vi "Sous_VI_recule.vi"   [LabVIEW 2017]
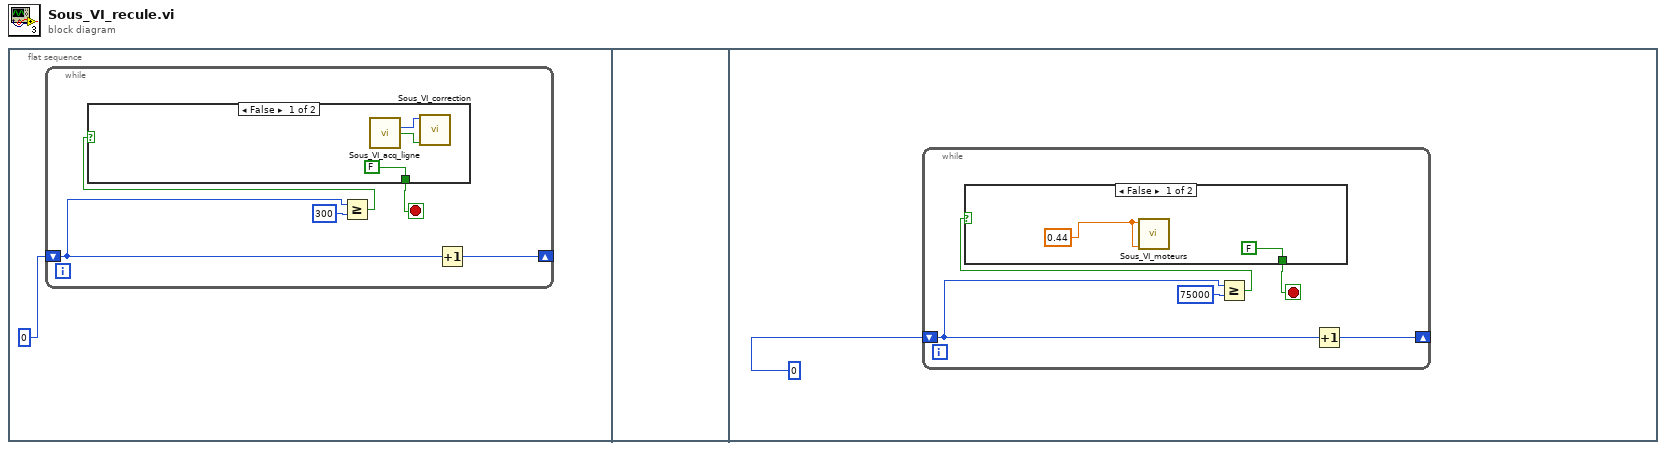
[diagram p0: block diagram]
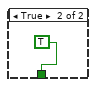
[diagram p2: hidden frame]
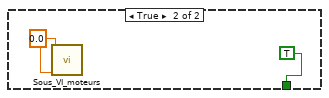
[diagram p3: hidden frame]
diagram:
  n1 = flat-sequence {
    frame #0 {
      n2 = while {
        shift-right: [w6] -> _
        shift-left: 0 -> [w3]
        stop <- w4 stop-if-true
        n3 = Greater Or Equal?(x=w3, y=300) -> (x >= y?=w5:bool)
        n4 = case shown="False" w5 {
          tunnel: [FALSE TRUE] -> w4
          frame False {
            n5 = call "Sous_VI_acq_ligne.vi"() -> ("Décalage"=w8:u32, "G/D ?"=w7:bool)  [unwired: 11 in, 3 out]
            n6 = call "Sous_VI_correction.vi"("G/D ?"=w7, "Décalage"=w8) -> ()  [unwired: 10 in]
          }
          frame True {
          }
        }
        n7 = Increment(x=w3) -> (x+1=w6:i32)
      }
    }
    frame #1 {
    }
    frame #2 {
      n8 = while {
        shift-right: [w16] -> _
        shift-left: 0 -> [w13]
        stop <- w14 stop-if-true
        n9 = Greater Or Equal?(x=w13, y=75000) -> (x >= y?=w15:bool)
        n10 = case shown="False" w15 {
          tunnel: [FALSE TRUE] -> w14
          frame False {
            w17 = 0.44 ("moteur gauche vite")
            n11 = call "Sous_VI_moteurs.vi"("Moteur Droit"=w17, "Moteur Gauche"=w17) -> ()  [unwired: 10 in]
          }
          frame True {
            w19 = 0.0 ("Moteur Gauche")
            n12 = call "Sous_VI_moteurs.vi"("Moteur Droit"=w19, "Moteur Gauche"=w19) -> ()  [unwired: 10 in]
          }
        }
        n13 = Increment(x=w13) -> (x+1=w16:i32)
      }
    }
  }
